vi "Day 19.vi"() -> ()   [LabVIEW 2021]
uses:
  a026a2ab-26f8-4a39-8e1d-061d06921e16.vi
  ec2ad6d2-8c51-4d9e-985b-4ec09321e157.vi
  <vilib>/Utility/file.llb/Read Delimited Spreadsheet (string).vi
panel:
  out "Scanner Positions Relative to Scanner 0":i32[][](array[numeric])
  out "Max Manhatten Distance (Part 2)":i32
  out "Number of Beacons":i32
  out "Input":string[](array[string])
  in  "Input File":enum32{"example input", "input"}(radio)
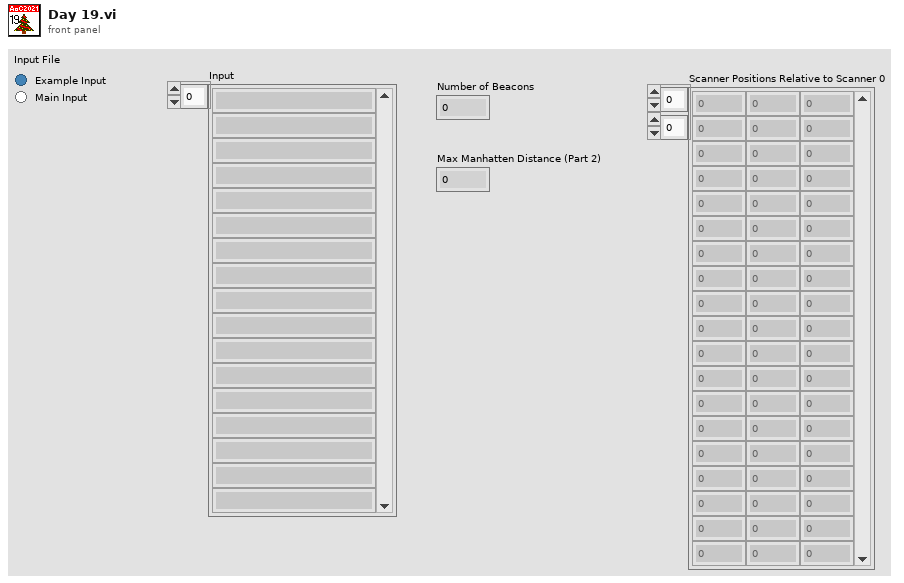
[diagram p1: front panel]
types:
  T1 = typedef "NI_Matrix.lvlib/RealMatrix.ctl" = dbl[][]
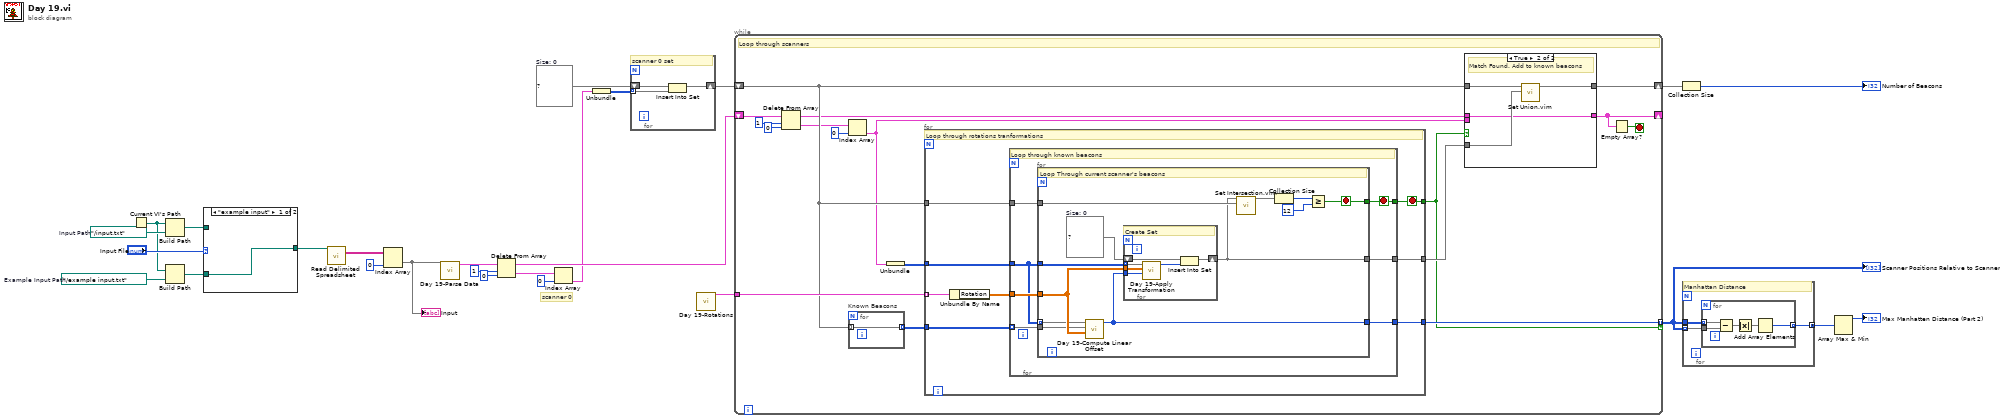
[diagram p0: block diagram]
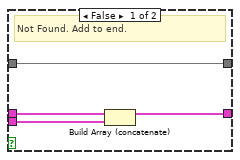
[diagram p2: hidden frame]
diagram:
  w12 = set{i32[]} {}  # Size: 0
  w25 = path "../example input.txt"  # Example Input Path
  w26 = path "../input.txt"  # Input Path
  # "scanner 0"
  n1 = Current VI's Path() -> (path=w20:path)
  n2 = Build Path(base path=w20, name or relative path=w26) -> (appended path=w23:path)
  n3 = Build Path(base path=w20, name or relative path=w25) -> (appended path=w22:path)
  n4 = case shown="\"example input\"" "Input File" {
    tunnel: w23 -> [_ w28]
    tunnel: w22 -> [w27 _]
    tunnel: [w27 w28] -> w21
    frame "example input" {
    }
    frame "input" {
    }
  }
  n5 = call-poly <vilib>:"Read Delimited Spreadsheet.vi"("file path (dialog if empty)"=w21) -> ("all rows"=w19:string[][])  [unwired: 9 in, 5 out]
  n6 = Index Array(array=w19, index (col)=0 ("disabled index (col)")) -> (element=w17:string[])  [unwired: 1 in]
  "Input" <- w17
  n7 = call "Day 19-Parse Data.vi"("Data in"=w17) -> ("Beacon Coordinate by Scanner"=w7:cluster{i32[][]}[])  [unwired: 10 in]
  n8 = Delete From Array(array=w7, length=1, index=0 ("index (page)")) -> (deleted portion=w11:cluster{i32[][]}[], array with subset deleted=w14:cluster{i32[][]}[])
  n9 = Index Array(array=w11, index=0 ("index (page)")) -> (element=w6:cluster{i32[][]})
  n10 = Unbundle(w6) -> (w5:i32[][])
  n11 = for {
    tunnel: w5 -> [w29] mode=indexing
    shift-right: [w31] -> w4
    shift-left: w12 -> [w30]
    # "scanner 0 set"
    n12 = Insert Into Set(10:w29, 11:w30) -> (3:w31:set{i32[]})  [unwired: 1 out]
  }
  n13 = call "Day 19-Rotations.vi"() -> ("Rotations"=w10:cluster{"Rotation":T1}[])  [unwired: 11 in]
  n14 = while {
    tunnel: w10 -> [w48]
    shift-right: [w46] -> w9
    shift-left: w4 -> [w44]
    shift-right: [w33] -> _
    shift-left: w14 -> [w43]
    tunnel: [w35] -> w3 mode=indexing if=w34
    stop <- w36 stop-if-true
    # "Loop through scanners"
    n15 = Delete From Array(array=w43, length=1, index=0) -> (deleted portion=w38:cluster{i32[][]}[], array with subset deleted=w40:cluster{i32[][]}[])
    n16 = Index Array(array=w38, index=0 ("index (page)")) -> (element=w37:cluster{i32[][]})
    n17 = for "Known Beacons" {
      tunnel: w44 -> [w82] mode=indexing
      tunnel: [w82] -> w45 mode=indexing
    }
    n18 = Unbundle(w37) -> (w32:i32[][])
    n19 = for {
      tunnel: w44 -> [w51]
      tunnel: w32 -> [w56]
      tunnel: w48 -> [w55] mode=indexing
      tunnel: [w53] -> w47
      tunnel: [w52] -> w35
      tunnel: w45 -> [w50]
      tunnel: [w49] -> w34
      stop <- w49 stop-if-true
      # "Loop through rotations tranformations"
      n20 = Unbundle By Name(w55) -> ("Rotation"=w54:T1)
      n21 = for {
        tunnel: w56 -> [w57]
        tunnel: w54 -> [w63]
        tunnel: w51 -> [w62]
        tunnel: [w61] -> w52
        tunnel: [w60] -> w53
        tunnel: [w59] -> w49
        tunnel: w50 -> [w58] mode=indexing
        stop <- w59 stop-if-true
        # "Loop through known beacons"
        n22 = for {
          tunnel: w63 -> [w68]
          tunnel: w62 -> [w75]
          tunnel: [w70] -> w61
          tunnel: [w74] -> w60
          tunnel: [w69] -> w59
          tunnel: w57 -> [w67]
          tunnel: w58 -> [w64]
          tunnel: w57 -> [w65] mode=indexing
          stop <- w69 stop-if-true
          w66 = set{i32[]} {}  # Size: 0
          # "Loop Through current scanner's beacons"
          n23 = call "Day 19-Compute Linear Offset.vi"("Rotation"=w68, "Reference Known Beacon"=w64, "Current Beacon Compare Point"=w65) -> ("Offset"=w70:i32[])  [unwired: 8 in]
          n24 = for {
            tunnel: w67 -> [w80] mode=indexing
            tunnel: w68 -> [w79]
            tunnel: w70 -> [w78]
            shift-right: [w76] -> w74
            shift-left: w66 -> [w81]
            # "Create Set"
            n25 = call "Day 19-Apply Transformation.vi"("3D LinearOffset"=w78, "Rotation"=w79, "Point in"=w80) -> ("Point out"=w77:i32[])  [unwired: 8 in]
            n26 = Insert Into Set(10:w77, 11:w81) -> (3:w76:set{i32[]})  [unwired: 1 out]
          }
          n27 = call "Set Intersection.vim"("set 2"=w75, "set 1"=w74) -> ("intersection"=w73:set{i32[]})  [unwired: 9 in]
          n28 = Collection Size(1:w73) -> (0:w72:i32)
          n29 = Greater Or Equal?(x=w72, y=12) -> (x >= y?=w69:bool)
        }
      }
    }
    n30 = case shown="True" w34 {
      tunnel: w47 -> [_ w90]
      tunnel: [w83 w89] -> w46
      tunnel: w44 -> [w83 w88]
      tunnel: w40 -> [w86 w87]
      tunnel: w37 -> [w85 _]
      tunnel: [w84 w87] -> w33
      frame False {
        # "Not Found. Add to end."
        n31 = Build Array (concatenate)(w86, w85) -> (w84:cluster{i32[][]}[])
      }
      frame True {
        # "Match Found. Add to known beacons"
        n32 = call "Set Union.vim"("set 2"=w90, "set 1"=w88) -> ("union"=w89:set{i32[]})  [unwired: 9 in]
      }
    }
    n33 = Empty Array?(array=w33) -> (empty?=w36:bool)
  }
  "Scanner Positions Relative to Scanner 0" <- w3
  n34 = Collection Size(1:w9) -> (0:→"Number of Beacons":i32)
  n35 = for {
    tunnel: w3 -> [w91] mode=indexing
    tunnel: [w93] -> w2 mode=concatenating
    tunnel: w3 -> [w92]
    # "Manhattan Distance"
    n36 = for {
      tunnel: w92 -> [w97] mode=indexing
      tunnel: w91 -> [w96]
      tunnel: [w98] -> w93 mode=indexing
      # "Manhattan Distance"
      n37 = Subtract(x=w97, y=w96) -> (x-y=w95:i32[])
      n38 = Absolute Value(x=w95) -> (abs(x)=w94:i32[])
      n39 = Add Array Elements(numeric array=w94) -> (sum=w98:i32)
    }
  }
  n40 = Array Max & Min(array=w2) -> (max value=→"Max Manhatten Distance (Part 2)":i32)  [unwired: 3 out]
